vi "Module Init.vi"(8 "error in (no error)":errorcluster, 11 "System Config Server in":refnum<class "System Config Module.lvclass">) -> (0 "error out":errorcluster, 3 "System Config Server out":refnum<class "System Config Module.lvclass">)   [LabVIEW 2020, in "Volatus.lvlib" / "System Config Module.lvclass"]
uses:
  System Config Module.lvclass
  System Config Module.lvclass/System Config Module.ctl
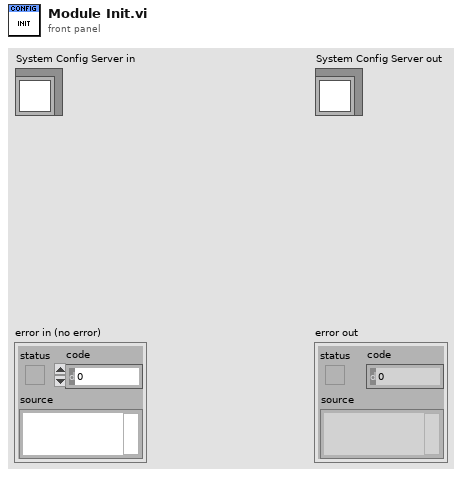
[diagram p1: front panel]
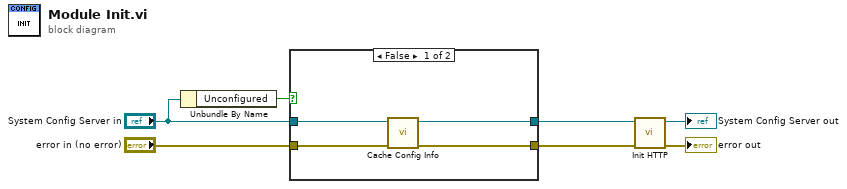
[diagram p0: block diagram]
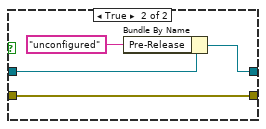
[diagram p2: hidden frame]
diagram:
  n1 = Unbundle By Name("System Config Server in") -> ("Unconfigured"=w1:bool)
  n2 = case shown="False" w1 {
    tunnel: "error in (no error)" -> [w11 w14]
    tunnel: [w10 w14] -> w6
    tunnel: [w9 w12] -> w3
    tunnel: "System Config Server in" -> [w8 w15]
    frame False {
      n3 = call "Cache Config Info.vi"("error in (no error)"=w11, "System Config Server in"=w8) -> ("error out"=w10:errorcluster, "System Config Server out"=w9:refnum<class "System Config Module.lvclass">)  [unwired: 8 in]
    }
    frame True {
      n4 = Bundle By Name(cluster=w15, "Pre-Release"="unconfigured") -> (w12:refnum<class "System Config Module.lvclass">)
    }
  }
  n5 = call "Init HTTP.vi"("error in (no error)"=w6, "System Config Server in"=w3) -> ("error out"=→"error out":errorcluster, "System Config Server out"=→"System Config Server out":refnum<class "System Config Module.lvclass">)  [unwired: 8 in]
